vi "readVisaMaybe.vi"(4 "Bit in":dbl, 5 "error in":errorcluster, 6 "VISA resource name in":refnum<visa-resource-name>, 7 "VISA connected?":bool) -> (0 "String Read":string, 1 "error out":errorcluster, 2 "VISA resource name out":refnum<visa-resource-name>)   [LabVIEW 2025]
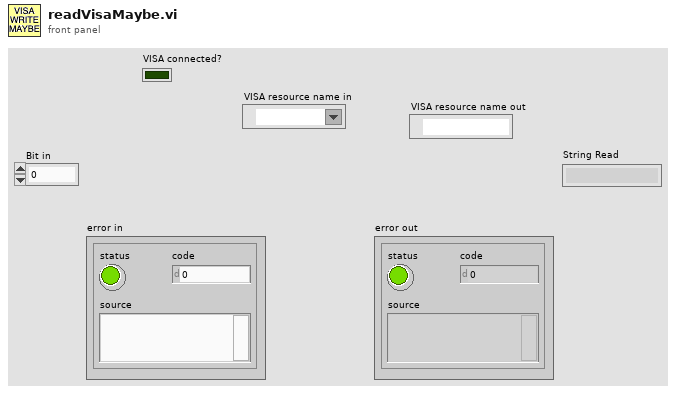
[diagram p1: front panel]
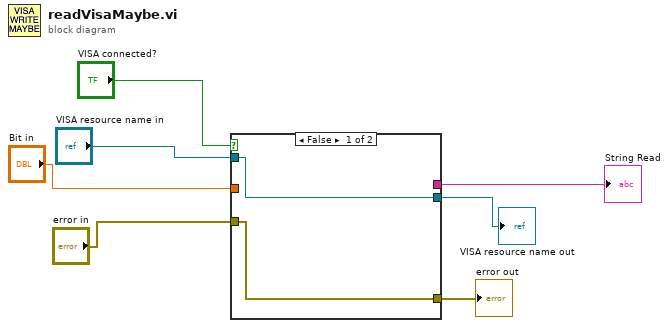
[diagram p0: block diagram]
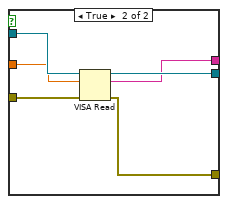
[diagram p2: hidden frame]
diagram:
  n1 = case shown="False" "VISA connected?" {
    tunnel: "VISA resource name in" -> [w9 w15]
    tunnel: "Bit in" -> [_ w14]
    tunnel: "error in" -> [w8 w13]
    tunnel: [w8 w12] -> w4
    tunnel: [w9 w11] -> w3
    tunnel: [_ w10] -> w1
    frame False {
    }
    frame True {
      n2 = VISA Read(VISA resource name=w15, byte count=w14, error in (no error)=w13) -> (VISA resource name out=w11:refnum<visa-resource-name>, read buffer=w10:string, error out=w12:errorcluster)  [unwired: 1 out]
    }
  }
  "String Read" <- w1
  "error out" <- w4
  "VISA resource name out" <- w3
